vi "TIcks per decisecond to Rotations per second.vi"(11 "Drive Velocities (ticks/ds)":T1) -> (3 "Drive Velocities (rotations/s)":T1)   [LabVIEW 2023]
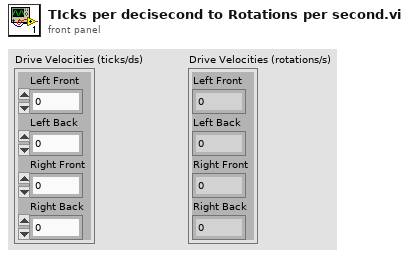
[diagram p1: front panel]
types:
  T1 = cluster{"Left Front":dbl, "Left Back":dbl, "Right Front":dbl, "Right Back":dbl}
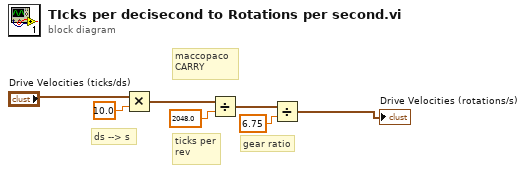
[diagram p0: block diagram]
diagram:
  # "ds --> s"
  # "ticks per\nrev"
  # "gear ratio"
  # "maccopaco\nCARRY"
  n1 = Multiply(x="Drive Velocities (ticks/ds)", y=10.0) -> (x*y=w3:T1)
  n2 = Divide(x=w3, y=2048.0) -> (x/y=w2:T1)
  n3 = Divide(x=w2, y=6.75) -> (x/y=→"Drive Velocities (rotations/s)":T1)
